vi "Init SelectionList.vi"(6 "Selection Mode":T1, 7 "ListSelection in":refnum<class "ListSelection.lvclass">, 8 "error in":errorcluster, 9 "Timeout (-1)":i32=-1, 10 "Items List":string[](array[string]), 11 "Message":string) -> (0 "error out":errorcluster, 3 "ListSelection out":refnum<class "ListSelection.lvclass">)   [LabVIEW 2012, in "ListSelection.lvlib" / "ListSelection.lvclass"]
doc: "Instantiates an object of class \"Error Message Box\"."
uses:
  ListSelection.lvclass
  Selection Mode.ctl
  ListSelection.lvclass/ListSelection.ctl
  MessageBox/MessageBox.lvclass
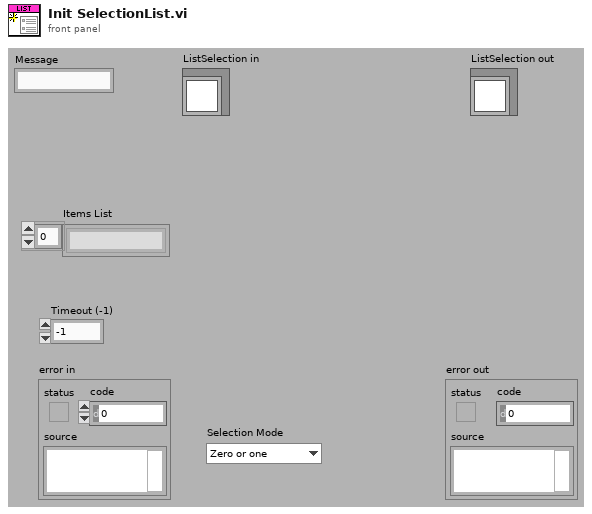
[diagram p1: front panel]
types:
  T1 = typedef "ListSelection.lvlib/ListSelection.lvclass/Selection Mode.ctl" = enum16{"Zero or one", "One", "Zero or more", "One or more"}
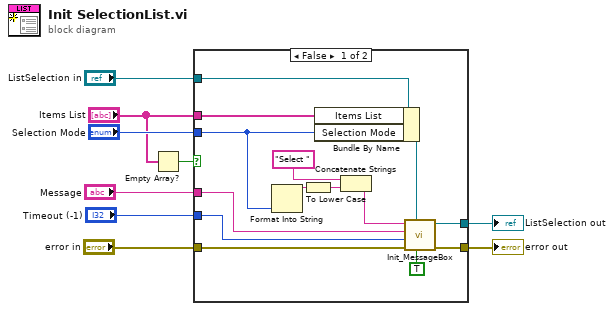
[diagram p0: block diagram]
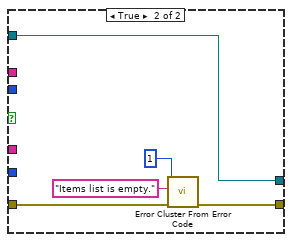
[diagram p2: hidden frame]
diagram:
  n1 = Empty Array?(array="Items List") -> (empty?=w1:bool)
  n2 = case shown="False" w1 {
    tunnel: "ListSelection in" -> [w23 w28]
    tunnel: [w21 w28] -> w8
    tunnel: "Timeout (-1)" -> [w20 _]
    tunnel: "error in" -> [w19 w27]
    tunnel: [w18 w26] -> w5
    tunnel: "Message" -> [w17 _]
    tunnel: "Selection Mode" -> [w14 _]
    tunnel: "Items List" -> [w15 _]
    frame False {
      n3 = Format Into String(w14) -> (resulting string=w12:string)  [unwired: 3 in, 1 out]
      n4 = To Lower Case(string=w12) -> (all lower case string=w11:string)
      n5 = Bundle By Name(cluster=w23, "Items List"=w15, "Selection Mode"=w14) -> (w22:refnum<class "ListSelection.lvclass">)
      n6 = Concatenate Strings("Select " ("MsgBox Title"), w11) -> (w10:string)
      n7 = call "Init_MessageBox.vi"("Allow to close? (T)"=TRUE, "MessageBox in"=w22, "error in (no error)"=w19, "Timeout (-1)"=w20, "Message"=w17, "MsgBox Title"=w10) -> ("error out"=w18:errorcluster, "MessageBox out"=w21:refnum<class "ListSelection.lvclass">)  [unwired: 1 in, 3 out]
    }
    frame True {
      n8 = call <vilib>:"Error Cluster From Error Code.vi"("error in (no error)"=w27, "error message (\"\")"="Items list is empty." ("error message (\"\")"), "error code (0)"=1) -> ("error out"=w26:errorcluster)  [unwired: 6 in]
    }
  }
  "ListSelection out" <- w8
  "error out" <- w5
